vi "Call Function with IMAQ Objects.vi"(8 "error in (no error)":errorcluster) -> (0 "error out":errorcluster)   [LabVIEW 2020]
uses:
  908d8fb0-7b42-46e8-9e96-a0c6d44c2c93.vi
  G-Embedded-Python-Interpreter-Toolkit-IMAQ/IMAQ to Py Object.vi/22f05568-5bba-4402-9e98-aca160827363.vi
  G-Embedded-Python-Interpreter-Toolkit/Null Py Object Refnum.vi
  908d8fb0-7b42-46e8-9e96-a0c6d44c2c93.vi/96ddca92-7bbf-40e2-a1a5-d32f291eb6af.vi
  G-Embedded-Python-Interpreter-Toolkit/Python Object Reference to Pointer Sized Ref.vi
  G-Embedded-Python-Interpreter-Toolkit/Pointer Sized Ref to Python Object Reference.vi
  G-Embedded-Python-Interpreter-Toolkit/Merge Call Library Errors.vi
  G-Embedded-Python-Interpreter-Toolkit/Create Py Object IMAQ Image.vi
  <vilib>/addons/_JKI Toolkits/Caraya/classes/Assert/Assert Not Error.vi
  G-Embedded-Python-Interpreter-Toolkit/Generate Argument Type Info.vi
  <vilib>/addons/_JKI Toolkits/Caraya/classes/Assert/Assert Equal Value and Type_Variant.vi
  G-Embedded-Python-Interpreter-Toolkit/G-Embedded-Python-Interpreter-Toolkit.lvlib
  <vilib>/addons/_JKI Toolkits/Caraya/classes/Test/Test.lvclass
  <vilib>/addons/_JKI Toolkits/Caraya/classes/Assert/Assert.lvclass
  G-Embedded-Python-Interpreter-Toolkit-IMAQ/G-Embedded-Python-Interpreter-Toolkit-IMAQ.lvlib
panel:
  out "Image":T1(plugin-control)
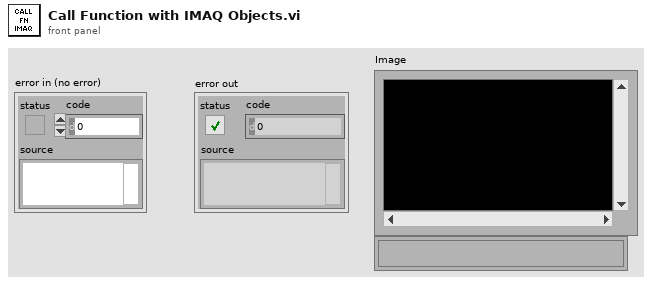
[diagram p1: front panel]
types:
  T1 = typedef "IMAQ Image.ctl" = refnum<image>
  T2 = cluster{"left":i16, "top":i16, "right":i16, "bottom":i16}
  T3 = typedef "Image Type" = u32
  T4 = typedef "imagedata.ctl" = cluster{"image type":i32, "image depth":i32, "image":u8[], "mask":u8[], "colors":u32[], "Rectangle":cluster{"left":i16, "top":i16, "right":i16, "bottom":i16}}
  T5 = typedef "G-Embedded-Python-Interpreter-Toolkit.lvlib/Python Object Reference.ctl" = refnum<k1>
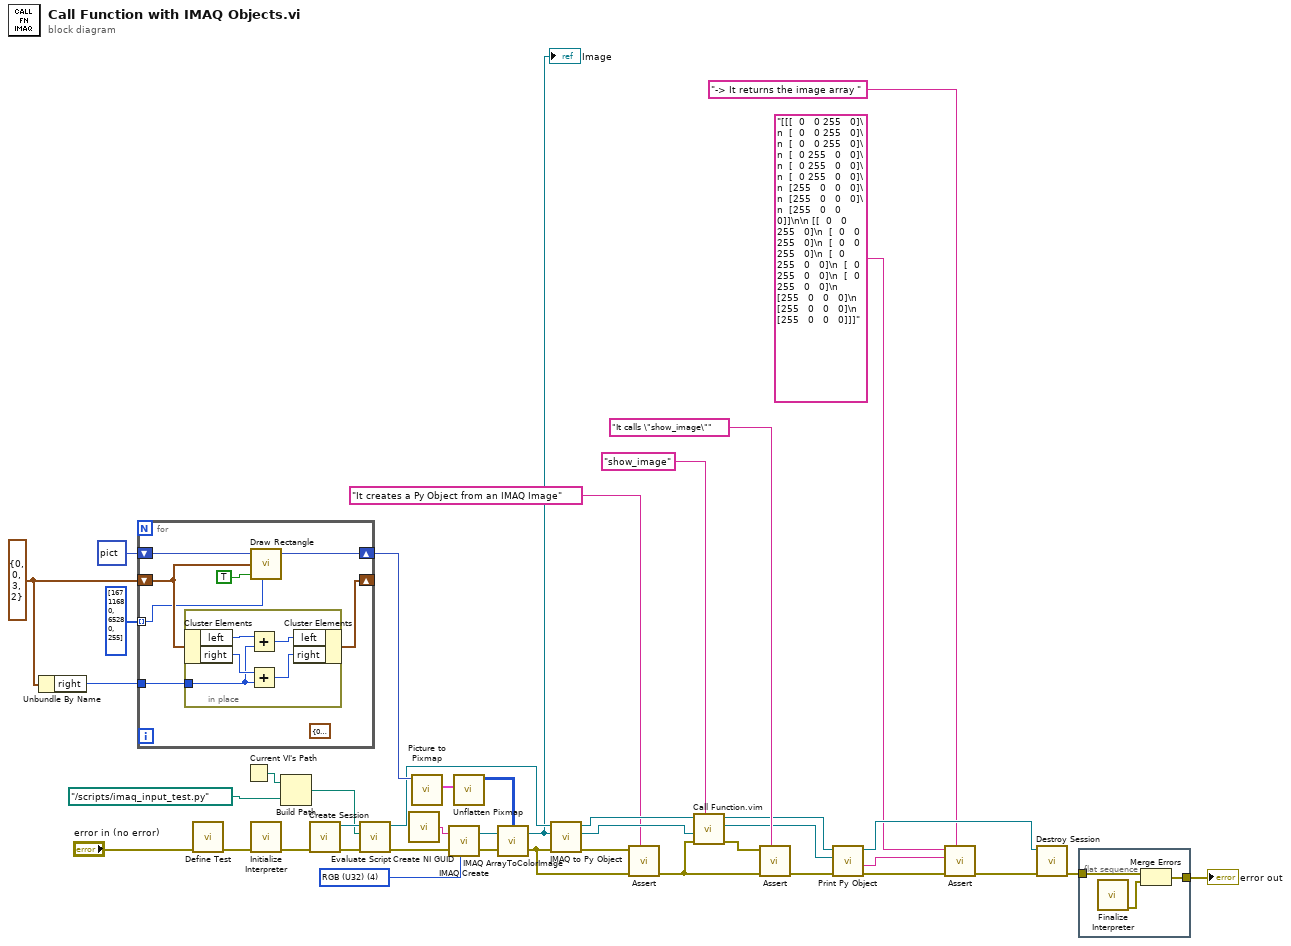
[diagram p0: block diagram]
diagram:
  w17 = T2 {"left"=0, "top"=0, "right"=3, "bottom"=2} ("rect")
  w28 = T3 4 items=["Grayscale (U8)", "Grayscale (I16)", "Grayscale (SGL)", "Complex (CSG)", "RGB (U32)", "HSL (U32)", "RGB (U64)", "Grayscale (U16)"] ("Image Type")
  n1 = Unbundle By Name(w17) -> ("right"=w16:i16)
  n2 = for {
    tunnel: u32[] [16711680, 65280, 255] ("color(black)") -> [w43] mode=indexing
    shift-right: [w48] -> w24
    shift-left: picture data[5B] ("new picture") -> [w47]
    shift-right: [w44] -> _
    shift-left: w17 -> [w46]
    tunnel: w16 -> [w45]
    (unwired) T2 {"left"=0, "top"=0, "right"=0, "bottom"=0} ("rect")
    n3 = in-place {
      in-place-border: w45 -> [w51]
      n4 = in-place-cluster #1(w46) -> ("left"=w54:i16, "right"=w52:i16)
      n5 = Add(x=w54, y=w51) -> (x+y=w53:i16)
      n6 = Add(x=w52, y=w51) -> (x+y=w50:i16)
      n7 = in-place-cluster #1("left"=w53, "right"=w50) -> (w44:T2)
    }
    n8 = call <vilib>:"Draw Rectangle.vi"("picture"=w47, "rect"=w46, "fill?(F)"=TRUE, "color(black)"=w43) -> ("new picture"=w48:picture)  [unwired: 5 in]
  }
  n9 = call <vilib>:"Define Test.vi"("error in (no error)"="error in (no error)") -> ("error out"=w42:errorcluster)  [unwired: 10 in]
  n10 = Current VI's Path() -> (path=w37:path)
  n11 = call "Initialize Interpreter.vi"("error in (no error)"=w42) -> ("error out"=w39:errorcluster)  [unwired: 9 in, 1 out]
  n12 = Build Path(base path=w37, name or relative path=path "../scripts/imaq_input_test.py" ("Path")) -> (appended path=w35:path)
  n13 = call "Create Session.vi"("error in (no error)"=w39) -> ("error out"=w34:errorcluster, "Session Handle"=w38:refnum<data-value>)  [unwired: 9 in]
  n14 = call "Evaluate Script.vi"("error in (no error)"=w34, "Script File Path"=w35, "Session Handle in"=w38) -> ("error out"=w22:errorcluster, "Session Handle out"=w20:refnum<data-value>)  [unwired: 7 in]
  n15 = call <vilib>:"Create NI GUID.vi"() -> ("NI GUID"=w27:string)
  n16 = call <vilib>:"Picture to Pixmap.vi"("picture"=w24) -> ("image data"=w23:T4)  [unwired: 9 in, 1 out]
  n17 = call "IMAQ Create"("Image Name"=w27, "Image Type"=w28, "error in (no error)"=w22) -> ("New Image"=w26:T1, "error out"=w21:errorcluster)  [unwired: 2 in]
  n18 = call <vilib>:"Unflatten Pixmap.vi"("image data"=w23) -> ("24-bit pixmap"=w25:u32[][])  [unwired: 4 in, 6 out]
  n19 = call "IMAQ ArrayToColorImage"("Image Pixels (U32)"=w25, "Image"=w26, "error in (no error)"=w21) -> ("Image Out"=w18:T1, "error out"=w3:errorcluster)  [unwired: 2 in]
  "Image" <- w18
  n20 = call "IMAQ to Py Object.vi"("error in (no error)"=w3, "Image In"=w18, "Session Handle in"=w20) -> ("error out"=w4:errorcluster, "Python Object Refnum"=w15:T5, "Session Handle out"=w19:refnum<data-value>)  [unwired: 6 in]
  n21 = call-poly <vilib>:"Assert.vi"("Label"="It creates a Py Object from an IMAQ Image", "error in (no error)"=w3, "Not Error?"=w4) -> ("error out"=w2:errorcluster)  [unwired: 8 in]
  n22 = call "Call Function.vim"("Function Name"="show_image", "error in (no error)"=w2, "Arguments in (Default - None)"=w15, "Data Value Reference in"=w19) -> ("error out"=w14:errorcluster, "Returned Python Object Refnum"=w8:T5, "Data Value Reference out"=w13:refnum<data-value>)  [unwired: 5 in]
  n23 = call-poly <vilib>:"Assert.vi"("Label"="It calls \"show_image\"", "error in (no error)"=w2, "Not Error?"=w14) -> ("error out"=w11:errorcluster)  [unwired: 8 in]
  n24 = call "Print Py Object.vi"("error in (no error)"=w11, "Python Object Refnum in"=w8, "Session Handle in"=w13) -> ("error out"=w10:errorcluster, "Print Ouptut"=w6:string, "Session Handle out"=w12:refnum<data-value>)  [unwired: 5 in, 1 out]
  n25 = call-poly <vilib>:"Assert.vi"("Label"="-> It returns the image array ", "error in (no error)"=w10, "Y"=w6, "X"="[[[  0   0 255   0]\n  [  0   0 255   0]\n  [  0   0 255   0]\n  [  0 255   0   0]\n  [  0 255   0   0]\n  [  0 255   0   0]\n  [255   0   0   0]\n  [255   0   0   0]\n  [255   0   0   0]]\n\n [[  0   0 255   0]\n  [  0   0 255   0]\n  [  0   0 255   0]\n  [  0 255   0   0]\n  [  0 255   0   0]\n  [  0 255   0   0]\n  [255   0   0   0]\n  [255   0   0   0]\n  [255   0   0   0]]]" ("Print Ouptut")) -> ("error out"=w9:errorcluster)  [unwired: 7 in]
  n26 = call "Destroy Session.vi"("error in (no error)"=w9, "Session Handle"=w12) -> ("error out"=w33:errorcluster)  [unwired: 9 in]
  n27 = flat-sequence {
    tunnel: w33 -> [w57]
    tunnel: [w55] -> w40
    frame #0 {
      n28 = call "Finalize Interpreter.vi"() -> ("error out"=w56:errorcluster)  [unwired: 11 in]
      n29 = Merge Errors(w57, w56) -> (w55:errorcluster)
    }
  }
  "error out" <- w40
